vi "RDV-autoscale.vi"(8 "error in (no error)":errorcluster, 10 "Autoscale":bool, 11 "RDV-Reflection_Data_viewer in":refnum<class "RDV-Reflection_Data_viewer.lvclass">) -> (0 "error out":errorcluster, 3 "RDV-Reflection_Data_viewer out":refnum<class "RDV-Reflection_Data_viewer.lvclass">)   [LabVIEW 2020, in "RDV-Reflection_Data_viewer.lvclass"]
doc: "Turns autoscale of the viewer's graphs on or off and refreshes them."
uses:
  RDV-Reflection_Data_viewer.lvclass
  RDV-Reflection_Data_viewer.lvclass/RDV-Reflection_Data_viewer.ctl
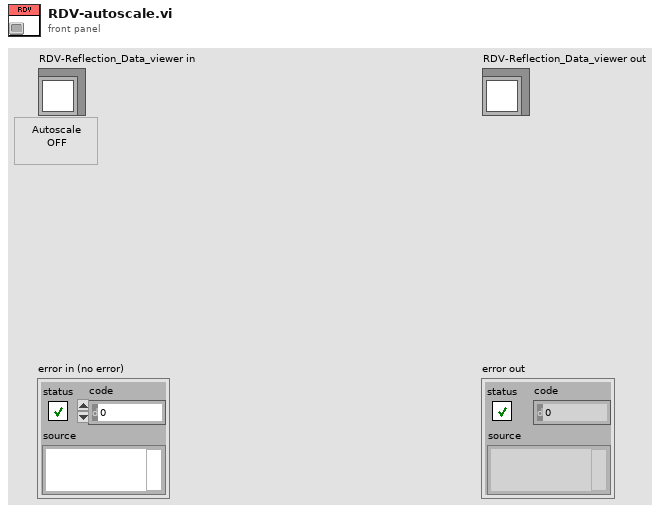
[diagram p1: front panel]
types:
  T1 = typedef "RDV-Reflection_Data_viewer.lvclass/RDV-XY_GRAPH_REFS.ctl" = cluster{"Reflection Real":refnum<vi>, "Reflection Imag":refnum<vi>, "Permittivity Real":refnum<vi>, "Permittivity Imag":refnum<vi>, "Impedance Real":refnum<vi>, "Impedance Imag":refnum<vi>}
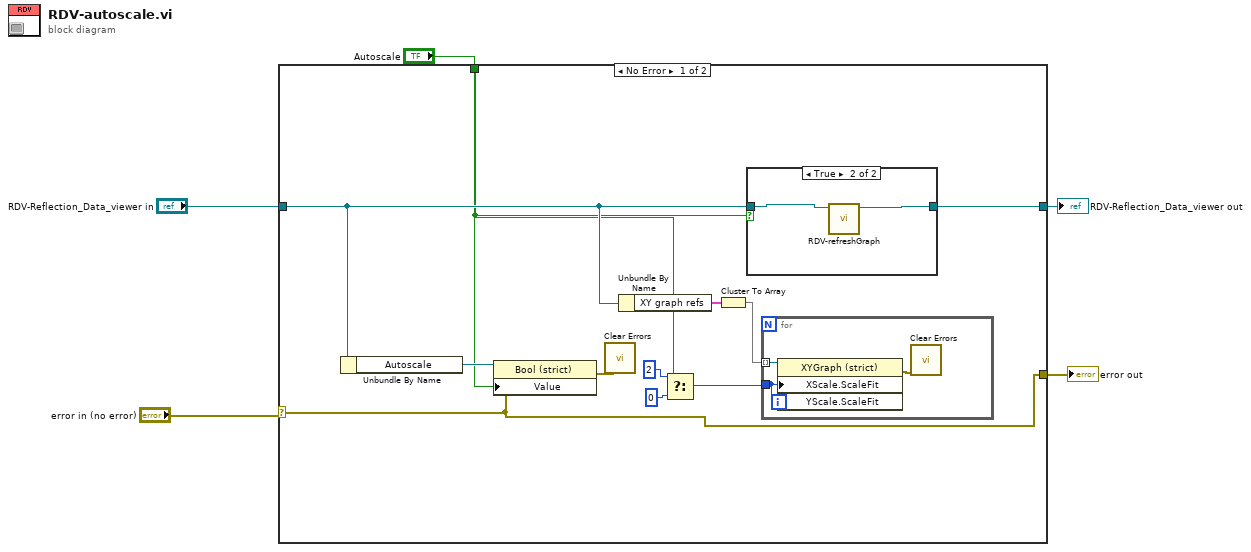
[diagram p0: block diagram]
diagram:
  n1 = case shown="No Error" "error in (no error)" {
    selector: "error in (no error)" -> [w6 w24]
    tunnel: [w6 w24] -> w4
    tunnel: [w7 w23] -> w2
    tunnel: "RDV-Reflection_Data_viewer in" -> [w9 w23]
    tunnel: "Autoscale" -> [w8 _]
    frame No Error {
      n2 = Unbundle By Name(w9) -> ("Autoscale"=w16:refnum<vi>)
      n3 = property class="Bool (strict)"(reference=w16, error in=w6, "Value"=w8) -> (error out=w10:errorcluster)  [unwired: 1 out]
      n4 = call <vilib>:"Clear Errors.vi"("error in (no error)"=w10) -> ()  [unwired: 5 in, 2 out]
      n5 = Unbundle By Name(w9) -> ("XY graph refs"=w15:T1)
      n6 = Select(t=u8 2 ("X Scale.Scale Fit"), s=w8, f=u8 0 ("X Scale.Scale Fit")) -> (s? t:f=w11:u8)
      n7 = Cluster To Array(cluster=w15) -> (array=w14:refnum<vi>[])
      n8 = case shown="True" w8 {
        tunnel: w9 -> [w17 w19]
        tunnel: [w17 w18] -> w7
        frame False {
        }
        frame True {
          n9 = call "RDV-refreshGraph.vi"("RDV-Reflection_Data_viewer in"=w19) -> ("RDV-Reflection_Data_viewer out"=w18:refnum<class "RDV-Reflection_Data_viewer.lvclass">)  [unwired: 9 in, 1 out]
        }
      }
      n10 = for {
        tunnel: w14 -> [w22] mode=indexing
        tunnel: w11 -> [w21]
        n11 = property class="XYGraph (strict)"(reference=w22, "XScale.ScaleFit"=w21, "YScale.ScaleFit"=w21) -> (error out=w20:errorcluster)  [unwired: 1 in, 1 out]
        n12 = call <vilib>:"Clear Errors.vi"("error in (no error)"=w20) -> ()  [unwired: 5 in, 2 out]
      }
    }
    frame Error {
    }
  }
  "error out" <- w4
  "RDV-Reflection_Data_viewer out" <- w2
